vi "SC Prepare Project.vi"(8 "error in (no error)":errorcluster, 10 "save VIs?":bool=TRUE) -> (0 "error out":errorcluster, 1 "project root":string, 2 "entry VI":path, 3 "ready?":bool, 4 "tool lines":string[](array[string]))   [LabVIEW 2023]
doc: "Common start of the Systemcore tools: finds the active project, optionally saves its modified VIs, runs systemcore-deploy info and, when the project isn't set up for deploys yet, offers to run systemcore-deploy init. Returns the project root, the entry VI, the info tool lines and whether to go on."
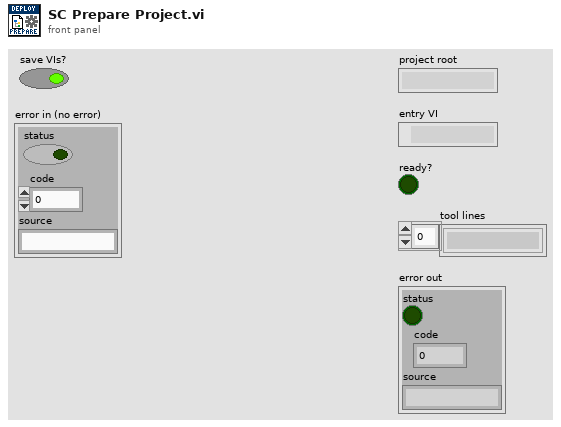
[diagram p1: front panel]
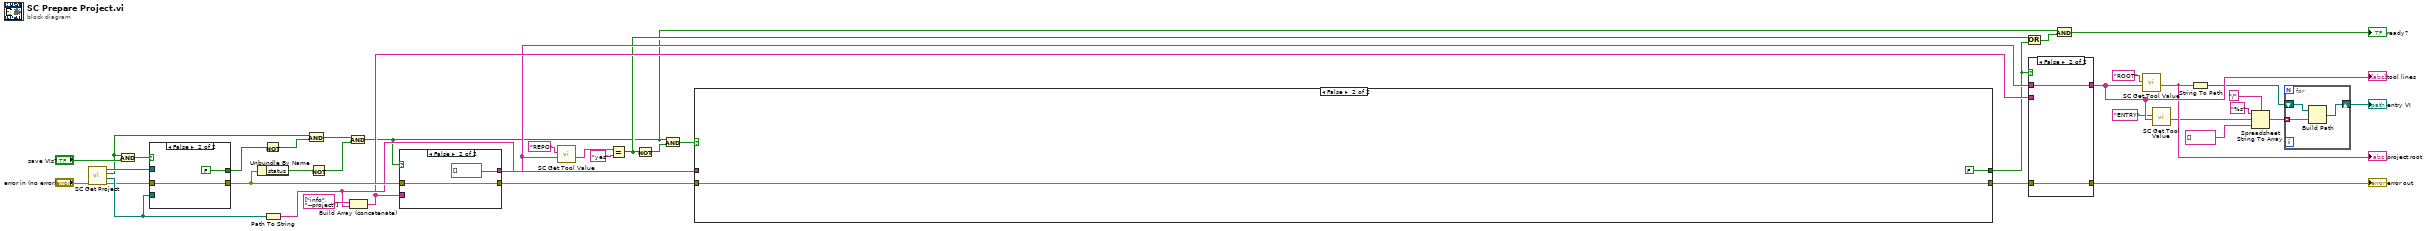
[diagram p0: block diagram]
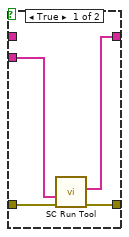
[diagram p2: hidden frame]
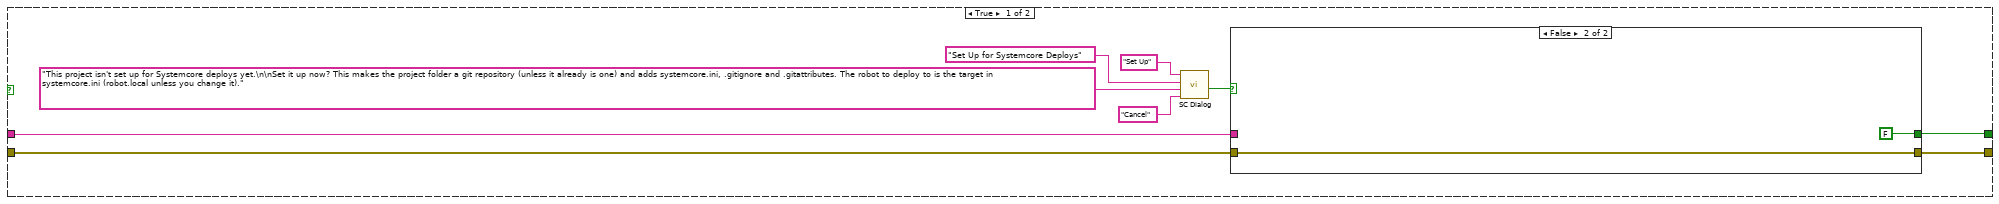
[diagram p3: hidden frame]
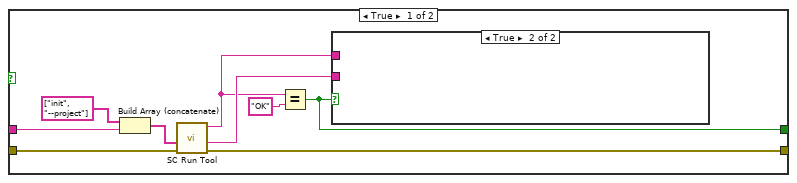
[diagram p4: hidden frame]
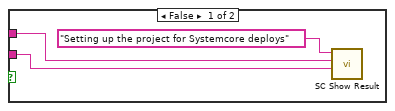
[diagram p5: hidden frame]
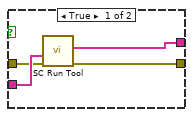
[diagram p6: hidden frame]
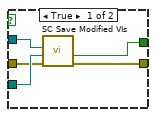
[diagram p7: hidden frame]
diagram:
  n1 = call <vilib>:"SC Get Project.vi"("error in (no error)"="error in (no error)") -> ("error out"=w37:errorcluster, "project folder"=w38:path, "found?"=w32:bool, "project application"=w36:refnum<vi>)  [unwired: 7 in]
  n2 = And(x=w32, y="save VIs?") -> (x .and. y?=w35:bool)
  n3 = case shown="False" w35 {
    tunnel: w38 -> [w46 _]
    tunnel: w37 -> [w44 w47]
    tunnel: w36 -> [w45 _]
    tunnel: [w43 FALSE] -> w34
    tunnel: [w42 w47] -> w28
    frame True {
      n4 = call <vilib>:"SC Save Modified VIs.vi"("error in (no error)"=w44, "project folder"=w46, "project application"=w45) -> ("error out"=w42:errorcluster, "cancelled?"=w43:bool)  [unwired: 7 in]
    }
    frame False {
    }
  }
  n5 = Unbundle By Name(w28) -> ("status"=w33:bool)
  n6 = Not(x=w34) -> (.not. x?=w31:bool)
  n7 = Path To String(path=w38) -> (string=w23:string)
  n8 = And(x=w32, y=w31) -> (x .and. y?=w30:bool)
  n9 = Not(x=w33) -> (.not. x?=w29:bool)
  n10 = And(x=w30, y=w29) -> (x .and. y?=w14:bool)
  n11 = Build Array (concatenate)(string[] ["info", "--project"], w23) -> (w20:string[])
  n12 = case shown="False" w14 {
    tunnel: w20 -> [w52 _]
    tunnel: w28 -> [w51 w53]
    tunnel: [w50 string[] []] -> w18
    tunnel: [w49 w53] -> w22
    frame True {
      n13 = call <vilib>:"SC Run Tool.vi"("error in (no error)"=w51, "arguments"=w52) -> ("error out"=w49:errorcluster, "tool lines"=w50:string[])  [unwired: 4 in, 4 out]
    }
    frame False {
    }
  }
  n14 = call <vilib>:"SC Get Tool Value.vi"("tool lines"=w18, "key"="REPO") -> ("value"=w26:string)  [unwired: 8 in, 1 out]
  n15 = Equal?(x=w26, y="yes") -> (x = y?=w16:bool)
  n16 = Not(x=w16) -> (.not. x?=w24:bool)
  n17 = And(x=w14, y=w24) -> (x .and. y?=w21:bool)
  n18 = case shown="False" w21 {
    tunnel: w23 -> [w59 _]
    tunnel: w22 -> [w58 w78]
    tunnel: [w56 FALSE] -> w15
    tunnel: [w55 w78] -> w19
    frame True {
      n19 = call "SC Dialog.vi"("Cancel text"="Cancel", "message"="This project isn't set up for Systemcore deploys yet.\n\nSet it up now? This makes the project folder a git repository (unless it already is one) and adds systemcore.ini, .gitignore and .gitattributes. The robot to deploy to is the target in systemcore.ini (robot.local unless you change it).", "window title"="Set Up for Systemcore Deploys", "OK text"="Set Up") -> ("OK?"=w57:bool)  [unwired: 7 in]
      n20 = case shown="False" w57 {
        tunnel: w59 -> [w71 _]
        tunnel: w58 -> [w69 w76]
        tunnel: [w65 FALSE] -> w56
        tunnel: [w64 w76] -> w55
        frame True {
          n21 = Build Array (concatenate)(string[] ["init", "--project"], w71) -> (w70:string[])
          n22 = call <vilib>:"SC Run Tool.vi"("error in (no error)"=w69, "arguments"=w70) -> ("error out"=w64:errorcluster, "output"=w67:string, "result"=w66:string)  [unwired: 4 in, 3 out]
          n23 = Equal?(x=w66, y="OK") -> (x = y?=w65:bool)
          n24 = case shown="True" w65 {
            tunnel: w67 -> [w75 _]
            tunnel: w66 -> [w74 _]
            frame False {
              n25 = call <vilib>:"SC Show Result.vi"("output"=w75, "result"=w74, "title"="Setting up the project for Systemcore deploys") -> ()  [unwired: 8 in, 1 out]
            }
            frame True {
            }
          }
        }
        frame False {
        }
      }
    }
    frame False {
    }
  }
  n26 = Or(x=w16, y=w15) -> (x .or. y?=w13:bool)
  n27 = case shown="False" w15 {
    tunnel: w20 -> [w83 _]
    tunnel: w19 -> [w82 w84]
    tunnel: w18 -> [_ w85]
    tunnel: [w81 w85] -> w10
    tunnel: [w80 w84] -> w17
    frame True {
      n28 = call <vilib>:"SC Run Tool.vi"("error in (no error)"=w82, "arguments"=w83) -> ("error out"=w80:errorcluster, "tool lines"=w81:string[])  [unwired: 4 in, 4 out]
    }
    frame False {
    }
  }
  "tool lines" <- w10
  "error out" <- w17
  n29 = And(x=w14, y=w13) -> (x .and. y?=→"ready?":bool)
  n30 = call <vilib>:"SC Get Tool Value.vi"("tool lines"=w10, "key"="ROOT") -> ("value"=w8:string)  [unwired: 8 in, 1 out]
  "project root" <- w8
  n31 = call <vilib>:"SC Get Tool Value.vi"("tool lines"=w10, "key"="ENTRY") -> ("value"=w6:string)  [unwired: 8 in, 1 out]
  n32 = String To Path(string=w8) -> (path=w1:path)
  n33 = Spreadsheet String To Array(delimiter (Tab)="/", format string="%s", spreadsheet string=w6, array type (2D Dbl)=string[] []) -> (array=w3:string[])
  n34 = for {
    tunnel: w3 -> [w87] mode=indexing
    shift-right: [w86] -> w2
    shift-left: w1 -> [w88]
    n35 = Build Path(base path=w88, name or relative path=w87) -> (appended path=w86:path)
  }
  "entry VI" <- w2
